vi "ACW ini file creation.vi"(0 "Ramp Time":string, 1 "ACW LO SET current value(mA)":string, 2 "ACW HI SET current value(mA)":string, 3 "ACW Test Time(S)":string, 4 "ACW Test Frequency(Hz)":string, 5 "error in (no error) 2":errorcluster, 6 "ACW voltage(kV)":string, 8 "configuration file path":path) -> (19 "error in (no error) 3":errorcluster)   [LabVIEW 2021]
uses:
  Template/Main_VI/Control/Ini.ctl
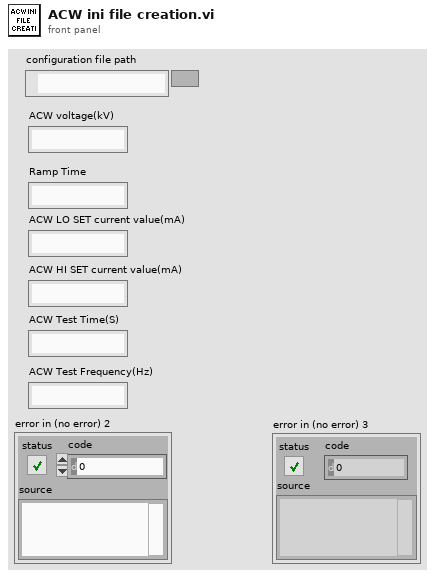
[diagram p1: front panel]
types:
  T1 = typedef "Ini.ctl" = enum16{"Write", "Read"}
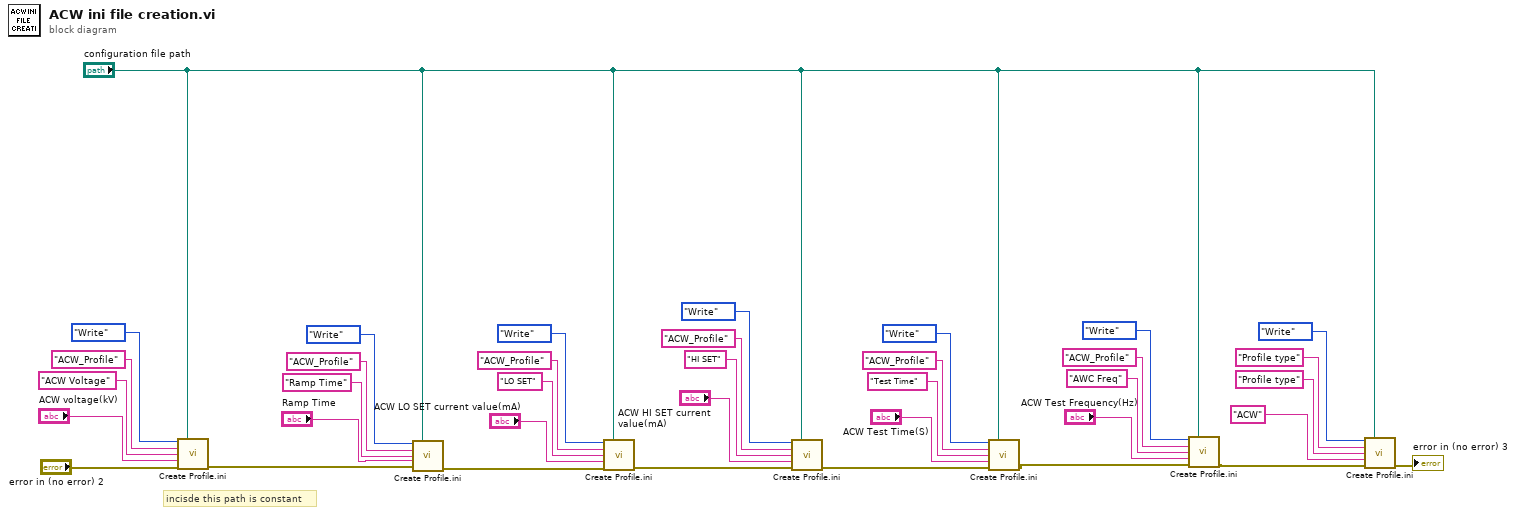
[diagram p0: block diagram]
diagram:
  # "incisde this path is constant"
  n1 = call "Create Profile.ini.vi"(0:Ini."Write", "configuration file path"="configuration file path", "Write Section"="ACW_Profile", "Write key"="ACW Voltage", "Write"="ACW voltage(kV)", "error in (no error)"="error in (no error) 2") -> ("error in (no error) 3"=w22:errorcluster)  [unwired: 8 in, 1 out]
  n2 = call "Create Profile.ini.vi"(0:Ini."Write", "configuration file path"="configuration file path", "Write Section"="ACW_Profile", "Write key"="Ramp Time", "Write"="Ramp Time", "error in (no error)"=w22) -> ("error in (no error) 3"=w21:errorcluster)  [unwired: 8 in, 1 out]
  n3 = call "Create Profile.ini.vi"(0:Ini."Write", "configuration file path"="configuration file path", "Write Section"="ACW_Profile", "Write key"="LO SET", "Write"="ACW LO SET current value(mA)", "error in (no error)"=w21) -> ("error in (no error) 3"=w20:errorcluster)  [unwired: 8 in, 1 out]
  n4 = call "Create Profile.ini.vi"(0:Ini."Write", "configuration file path"="configuration file path", "Write Section"="ACW_Profile", "Write key"="HI SET", "Write"="ACW HI SET current value(mA)", "error in (no error)"=w20) -> ("error in (no error) 3"=w19:errorcluster)  [unwired: 8 in, 1 out]
  n5 = call "Create Profile.ini.vi"(0:Ini."Write", "configuration file path"="configuration file path", "Write Section"="ACW_Profile", "Write key"="Test Time", "Write"="ACW Test Time(S)", "error in (no error)"=w19) -> ("error in (no error) 3"=w14:errorcluster)  [unwired: 8 in, 1 out]
  n6 = call "Create Profile.ini.vi"(0:Ini."Write", "configuration file path"="configuration file path", "Write Section"="ACW_Profile", "Write key"="AWC Freq", "Write"="ACW Test Frequency(Hz)", "error in (no error)"=w14) -> ("error in (no error) 3"=w9:errorcluster)  [unwired: 8 in, 1 out]
  n7 = call "Create Profile.ini.vi"(0:Ini."Write", "configuration file path"="configuration file path", "Write Section"="Profile type", "Write key"="Profile type", "Write"="ACW", "error in (no error)"=w9) -> ("error in (no error) 3"=→"error in (no error) 3":errorcluster)  [unwired: 8 in, 1 out]
